vi "Interpolator_Yuhe.vi"(10 "interpolation distance":dbl, 11 "Array in":cluster{"X":dbl, "Y":dbl}[](array[cluster])) -> (3 "Array out":cluster{"X":dbl, "Y":dbl}[](array[cluster]))   [LabVIEW 2019]
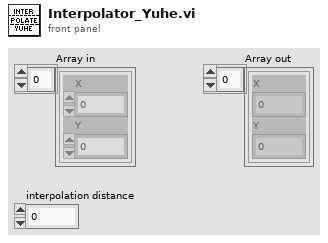
[diagram p1: front panel]
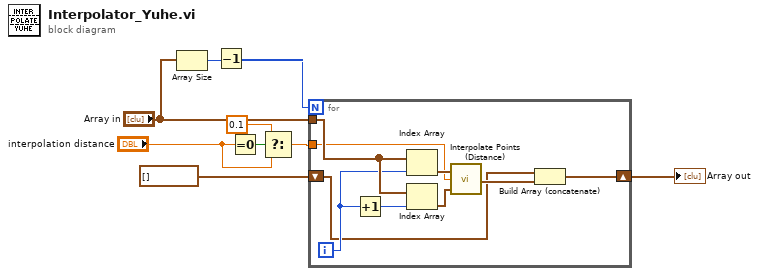
[diagram p0: block diagram]
diagram:
  n1 = Array Size(array="Array in") -> (size(s)=w7:i32)
  n2 = Decrement(x=w7) -> (x-1=w5:i32)
  n3 = Equal To 0?(x="interpolation distance") -> (x = 0?=w4:bool)
  n4 = Select(t=0.1, s=w4, f="interpolation distance") -> (s? t:f=w1:dbl)
  n5 = for {
    N: w5 -> [_]
    tunnel: "Array in" -> [w18]
    tunnel: w1 -> [w13]
    shift-right: [w11] -> w8
    shift-left: cluster{"X":dbl, "Y":dbl}[] [] -> [w10]
    i -> [w17]
    n6 = Increment(x=w17) -> (x+1=w16:i32)
    n7 = Index Array(array=w18, index=w17) -> (element=w15:cluster{"X":dbl, "Y":dbl})
    n8 = Index Array(array=w18, index=w16) -> (element=w14:cluster{"X":dbl, "Y":dbl})
    n9 = call "Interpolate Points (Distance).vi"("End Point"=w14, "Distance between Points"=w13, "Start Point"=w15) -> ("Output Point Array"=w12:cluster{"X":dbl, "Y":dbl}[])
    n10 = Build Array (concatenate)(w10, w12) -> (w11:cluster{"X":dbl, "Y":dbl}[])
  }
  "Array out" <- w8
